vi "get.vi"(10 "variables":string[](array[string])=["intout", "stringout", "time"], 11 "Experience ID":string="Test") -> (0 "error out":errorcluster={"status"=TRUE, "code"=1, "source"="Entry not found"}, 2 "values":string[](array[string])=["0"], 3 "names":string[](array[string])=["intout"])   [LabVIEW 2015]
panel:
  # "Get"
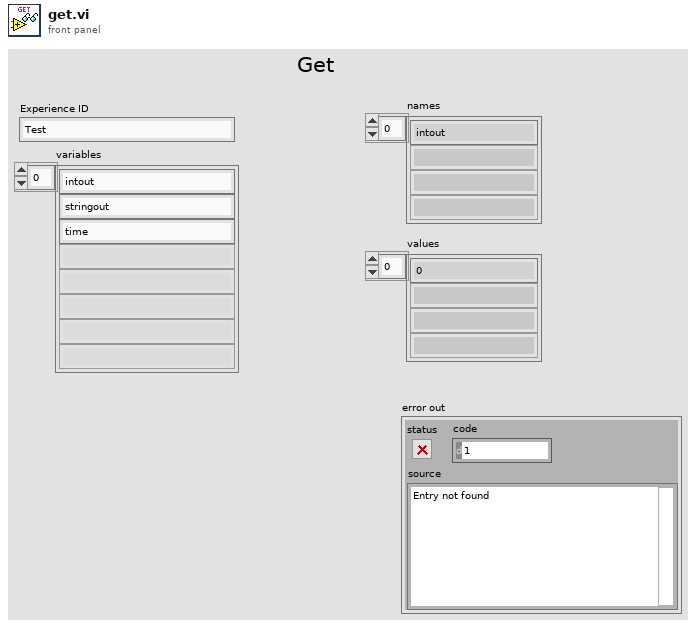
[diagram p1: front panel]
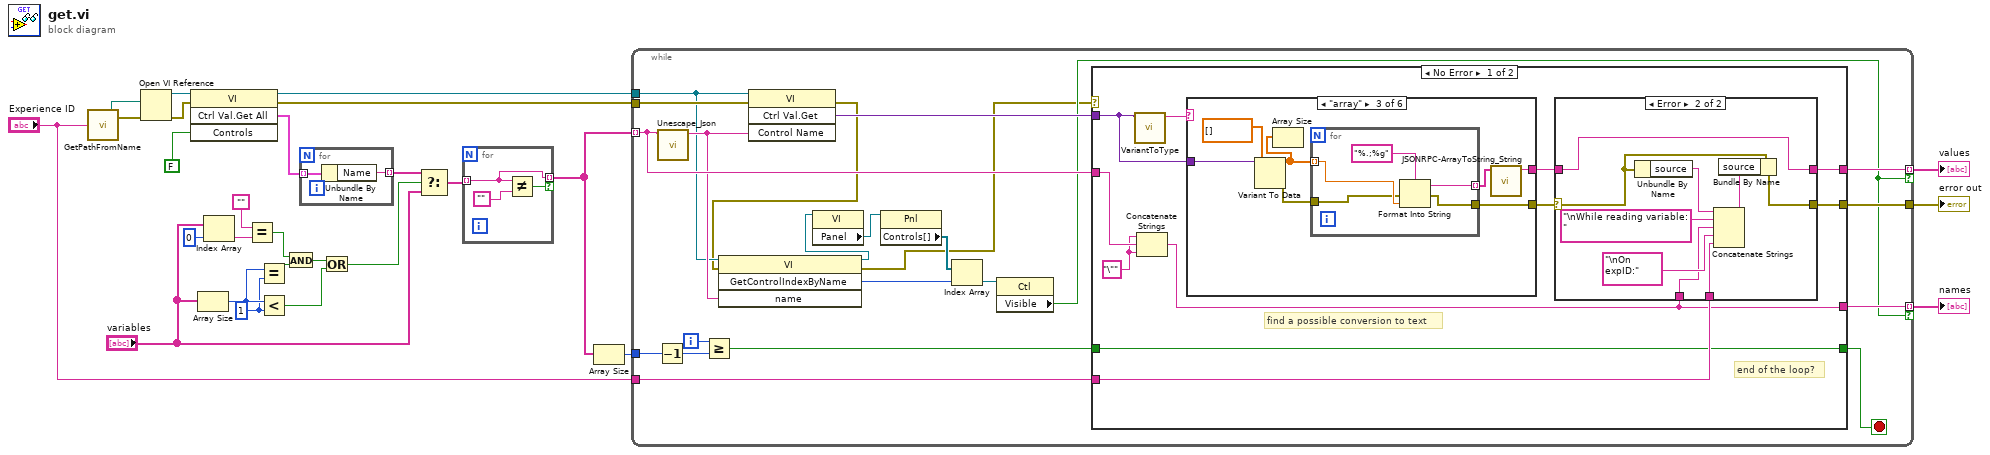
[diagram p0: block diagram]
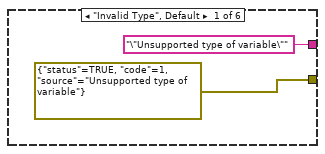
[diagram p3: hidden frame]
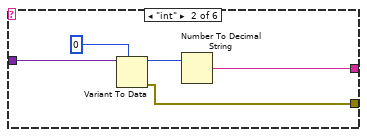
[diagram p4: hidden frame]
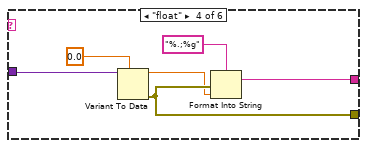
[diagram p5: hidden frame]
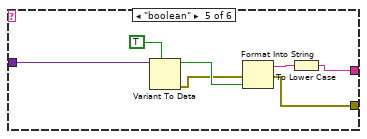
[diagram p6: hidden frame]
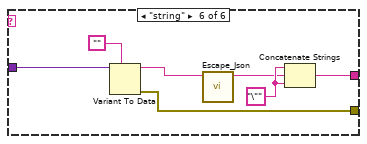
[diagram p7: hidden frame]
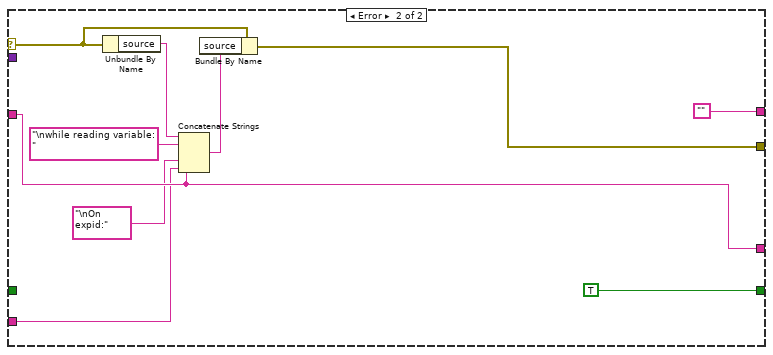
[diagram p8: hidden frame]
diagram:
  w13 = 1 ("y")
  n1 = call "GetPathFromName.vi"("Experience ID"="Experience ID") -> ("Error out"=w26:errorcluster, "VI_Path"=w27:path)
  n2 = Open VI Reference(vi path=w27, error in (no error)=w26) -> (vi reference=w20:refnum<vi>, error out=w10:errorcluster)  [unwired: 1 in, 3 out]
  n3 = invoke class="VI" method="Ctrl Val.Get All"(reference=w20, error in=w10, "Controls"=FALSE) -> (reference out=w19:refnum<vi>, error out=w9:errorcluster, "Get All Control Values Variant"=w17:cluster{"Name":string, "Variant Data":variant}[])  [unwired: 1 in, 1 out]
  n4 = Array Size(array="variables") -> (size(s)=w14:i32)
  n5 = Index Array(array="variables", index=0) -> (element=w4:string)
  n6 = Equal?(x="", y=w4) -> (x = y?=w7:bool)
  n7 = Equal?(x=w14, y=w13) -> (x = y?=w11:bool)
  n8 = Less?(x=w14, y=w13) -> (x < y?=w15:bool)
  n9 = And(x=w7, y=w11) -> (x .and. y?=w12:bool)
  n10 = for {
    tunnel: w17 -> [w29] mode=indexing
    tunnel: [w28] -> w16 mode=indexing
    n11 = Unbundle By Name(w29) -> ("Name"=w28:string)
  }
  n12 = Or(x=w12, y=w15) -> (x .or. y?=w3:bool)
  n13 = Select(t=w16, s=w3, f="variables") -> (s? t:f=w2:string[])
  n14 = for {
    tunnel: w2 -> [w31] mode=indexing
    tunnel: [w31] -> w1 mode=indexing if=w30
    n15 = Not Equal?(x=w31, y="") -> (x != y?=w30:bool)
  }
  n16 = Array Size(array=w1) -> (size(s)=w25:i32)
  n17 = while {
    tunnel: w1 -> [w43] mode=indexing
    tunnel: w19 -> [w38]
    tunnel: w25 -> [w47]
    tunnel: w9 -> [w54]
    tunnel: [w51] -> w21
    tunnel: [w50] -> w24 mode=indexing if=w35
    tunnel: [w49] -> w23 mode=indexing if=w35
    tunnel: "Experience ID" -> [w48]
    i -> [w45]
    stop <- w52 stop-if-true
    n18 = Decrement(x=w47) -> (x-1=w44:i32)
    n19 = call "Unescape_Json.vi"("Json_String"=w43) -> ("String"=w39:string)  [unwired: 9 in]
    n20 = Greater Or Equal?(x=w45, y=w44) -> (x >= y?=w46:bool)
    n21 = invoke class="VI" method="Ctrl Val.Get"(reference=w38, error in=w54, "Control Name"=w39) -> (error out=w34:errorcluster, "Get Control Value Variant"=w53:variant)  [unwired: 1 in, 2 out]
    n22 = invoke class="VI" method="GetControlIndexByName"(reference=w38, error in=w34, "name"=w39) -> (reference out=w36:refnum<vi>, error out=w33:errorcluster, "GetControlIndexByName"=w42:i32)  [unwired: 1 in, 1 out]
    n23 = property class="VI"(reference=w36) -> ("Panel"=w37:refnum<vi>)  [unwired: 1 in, 2 out]
    n24 = property class="Pnl"(reference=w37) -> ("Controls[]"=w41:refnum<vi>[])  [unwired: 1 in, 2 out]
    n25 = Index Array(array=w41, index=w42) -> (element=w40:refnum<vi>)
    n26 = property class="Ctl"(reference=w40) -> ("Visible"=w35:bool)  [unwired: 1 in, 2 out]
    n27 = case shown="No Error" w33 {
      selector: w33 -> [_ w124]
      tunnel: w53 -> [w57 _]
      tunnel: w46 -> [w55 _]
      tunnel: [w55 TRUE] -> w52
      tunnel: w43 -> [w59 w119]
      tunnel: [w64 w120] -> w51
      tunnel: [w62 ""] -> w50
      tunnel: [w60 w119] -> w49
      tunnel: w48 -> [w61 w116]
      frame No Error {
        w58 = "\"" ("string")
        # "end of the loop?"
        # "find a possible conversion to text"
        n28 = call "VariantToType.vi"("Variant"=w57) -> ("type Name"=w56:string)  [unwired: 10 in]
        n29 = Concatenate Strings(w58, w59, w58) -> (w60:string)
        n30 = case shown="\"array\"" w56 {
          tunnel: w57 -> [_ w82 w90 w100 w106 w114]
          tunnel: ["\"Unsupported type of variable\"" w80 w85 w96 w102 w111] -> w63
          tunnel: [errorcluster {"status"=TRUE, "code"=1, "source"="Unsupported type of variable"} ("error out") w79 w86 w99 w104 w113] -> w65
          frame "Invalid Type", Default {
          }
          frame "int" {
            n31 = Variant To Data(type=0, Variant=w82) -> (data=w81:i32, error out=w79:errorcluster)  [unwired: 1 in]
            n32 = Number To Decimal String(number=w81) -> (decimal integer string=w80:string)  [unwired: 1 in]
          }
          frame "array" {
            n33 = Variant To Data(type=dbl[] [] ("Array"), Variant=w90) -> (data=w88:dbl[], error out=w87:errorcluster)  [unwired: 1 in]
            n34 = Array Size(array=w88) -> ()  [unwired: 1 out]
            n35 = for {
              tunnel: w88 -> [w94] mode=indexing
              tunnel: w87 -> [w93]
              tunnel: [w92] -> w86
              tunnel: [w91] -> w84 mode=indexing
              n36 = Format Into String(format string="%.;%g", error in=w93, w94) -> (resulting string=w91:string, error out=w92:errorcluster)  [unwired: 1 in]
            }
            n37 = call "JSONRPC-ArrayToString_String.vi"("Array"=w84) -> ("Output"=w85:string)  [unwired: 10 in]
          }
          frame "float" {
            n38 = Variant To Data(type=0.0, Variant=w100) -> (data=w98:dbl, error out=w99:errorcluster)  [unwired: 1 in]
            n39 = Format Into String(format string="%.;%g", error in=w99, w98) -> (resulting string=w96:string)  [unwired: 1 in, 1 out]
          }
          frame "boolean" {
            n40 = Variant To Data(type=TRUE, Variant=w106) -> (data=w108:bool, error out=w107:errorcluster)  [unwired: 1 in]
            n41 = Format Into String(error in=w107, w108) -> (resulting string=w103:string, error out=w104:errorcluster)  [unwired: 2 in]
            n42 = To Lower Case(string=w103) -> (all lower case string=w102:string)
          }
          frame "string" {
            w112 = "\"" ("string")
            n43 = Variant To Data(type="", Variant=w114) -> (data=w109:string, error out=w113:errorcluster)  [unwired: 1 in]
            n44 = call "Escape_Json.vi"("String"=w109) -> ("Json_string"=w110:string)  [unwired: 9 in]
            n45 = Concatenate Strings(w112, w110, w112) -> (w111:string)
          }
        }
        n46 = case shown="Error" w65 {
          selector: w65 -> [w67 w75]
          tunnel: [w67 w76] -> w64
          tunnel: [w66 w68] -> w62
          tunnel: w63 -> [w66 w68]
          tunnel: w60 -> [_ w70]
          tunnel: w61 -> [_ w69]
          frame No Error {
            # "add to the list"
          }
          frame Error {
            n47 = Unbundle By Name(w75) -> ("source"=w74:string)
            n48 = Concatenate Strings(w74, "\nWhile reading variable: " ("string"), w70, "\nOn expID:" ("string"), w69) -> (w72:string)
            n49 = Bundle By Name(cluster=w75, "source"=w72) -> (w76:errorcluster)
          }
        }
      }
      frame Error {
        n50 = Unbundle By Name(w124) -> ("source"=w123:string)
        n51 = Concatenate Strings(w123, "\nwhile reading variable: " ("string"), w119, "\nOn expid:", w116) -> (w121:string)
        n52 = Bundle By Name(cluster=w124, "source"=w121) -> (w120:errorcluster)
      }
    }
  }
  "error out" <- w21
  "names" <- w23
  "values" <- w24
